vi "RichToFlatbackend_response.vi"(5 "OutputClusterType":T1, 11 "InputCluster":T2) -> (3 "OutputCluster":T1)   [LabVIEW 2020, in "lexitekDriver_client.lvlib"]
uses:
  lexitekDriver_client.lvlib
  backend_response.ctl
  backend_response_Flat.ctl
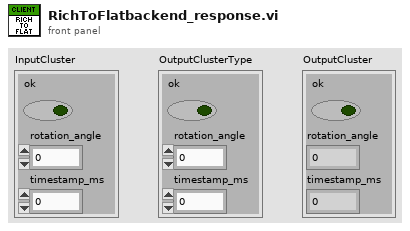
[diagram p1: front panel]
types:
  T1 = typedef "lexitekDriver_client.lvlib/backend_response_Flat.ctl" = cluster{"ok":bool, "rotation_angle":dbl, "timestamp_ms":u64}
  T2 = typedef "lexitekDriver_client.lvlib/backend_response.ctl" = cluster{"ok":bool, "rotation_angle":dbl, "timestamp_ms":u64}
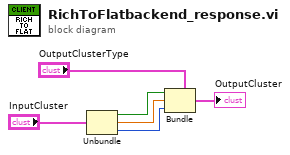
[diagram p0: block diagram]
diagram:
  n1 = Unbundle "Unbundle"("InputCluster") -> ("ok"=w3:bool, "rotation_angle"=w2:dbl, "timestamp_ms"=w1:u64)
  n2 = Bundle "Bundle"(cluster="OutputClusterType", "ok"=w3, "rotation_angle"=w2, "timestamp_ms"=w1) -> (→"OutputCluster":T1)
